vi "Tools Dialog.vi"(7 "Settings":T1, 8 "Error In":errorcluster, 10 "Context":refnum<k7>, 11 "Tools In":refnum<class "Tools.lvclass">[](array[class])) -> (0 "Error Out":errorcluster, 1 "Canceled?":bool, 2 "ID":string, 3 "Tools Out":refnum<class "Tools.lvclass">[](array[class]))   [LabVIEW 2021, in "Seq Edit Quick Drop.lvlib"]
uses:
  Seq Edit Quick Drop.lvlib
  Resources/Tool Menu Utility.lvlibp/Tools/Tools.lvclass
  Control Keys.ctl
  Get Modifier.vi
  <vilib>/addons/TestStand/_TSUtility.llb/TestStand - Start Modal Dialog (Sequence Context).vi
  <vilib>/Utility/error.llb/Trim Whitespace.vi
  <vilib>/addons/TestStand/_TSUtility.llb/TestStand - End Modal Dialog (Sequence Context).vi
panel:
  in  "Parameters":string
  in  "Tools":string(tree)
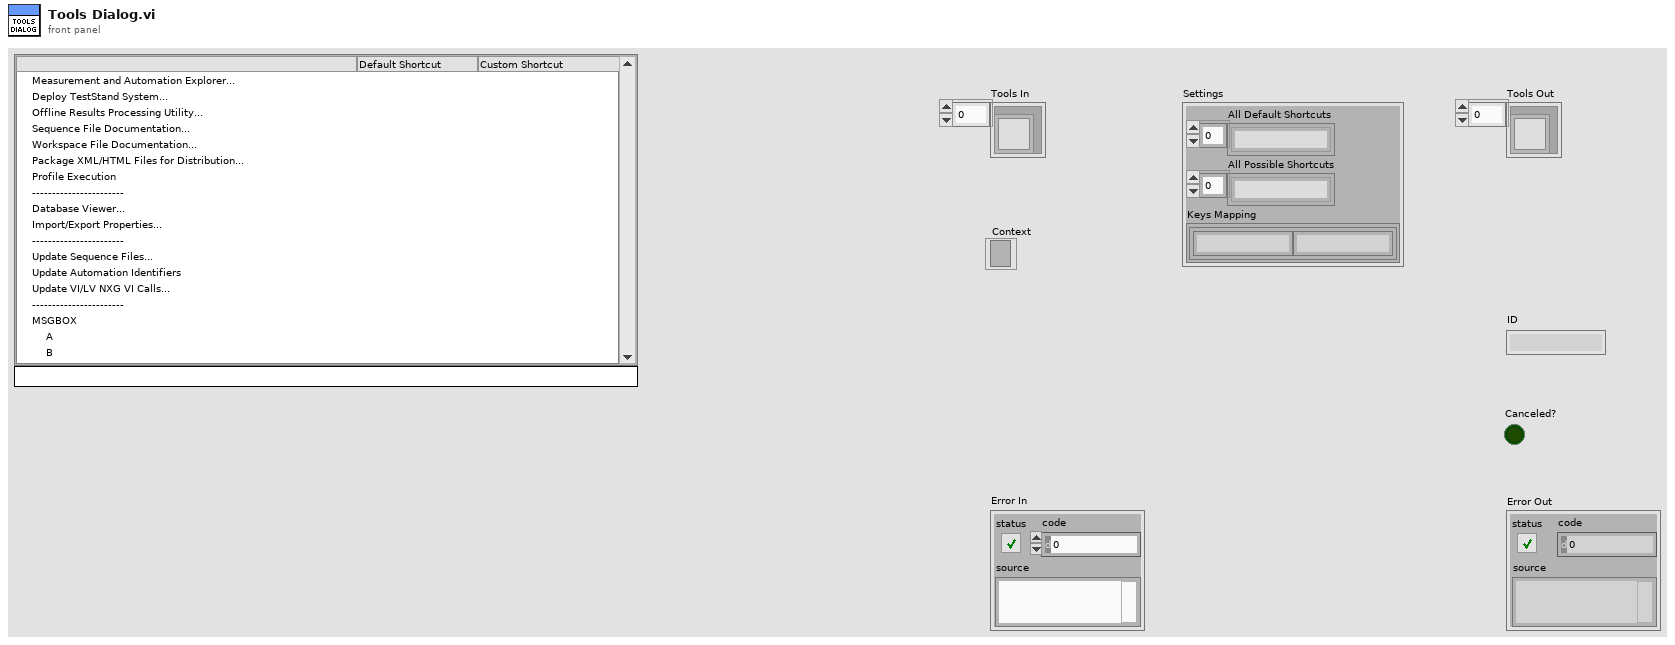
[diagram p1: front panel]
types:
  T1 = cluster{"All Default Shortcuts":string[], "All Possible Shortcuts":string[], "Keys Mapping":map{string, string}}
  T2 = typedef "Seq Edit Quick Drop.lvlib/Control Keys.ctl" = enum16{"Other", "Enter", "Escape", "Tab", "Up", "Down"}
  T3 = typedef "TestStand - Status Monitor.ctl" = cluster{"Sequence Context":refnum<k7>, "Execution":refnum<k7>, "Termination Monitor":refnum<k7>}
  T4 = cluster{"Shift":bool, "Ctrl":bool, "Alt":bool, "Cmd":bool, "Opt":bool}
  T5 = typedef "eventvkey.ctl" = enum16{"ASCII", "Enter", "Return", "Shift", "Ctrl", "Alt", "Cmd", "Opt", "Caps", "NumLock", "Clear", "Break", "Up", "Down", "Left", "Right", "Insert", "Delete", "Home", "End", "PageUp", "PageDown", "Escape", "Help", "Pause", "ScrollLock", "F1", "F2", "F3", "F4", "F5", "F6", "F7", "F8", "F9", "F10", "F11", "F12", "F13", "F14", "F15", "F16", "F17", "F18", "F19", "F20", "F21", "F22", "F23", "F24", "Play", "VolumeUp", "VolumeDown", "Mute", "Two Byte Char"}
  T6 = typedef "Seq Edit Quick Drop.lvlib/Modifiers.ctl" = enum16{"SHIFT", "CTRL", "ALT"}
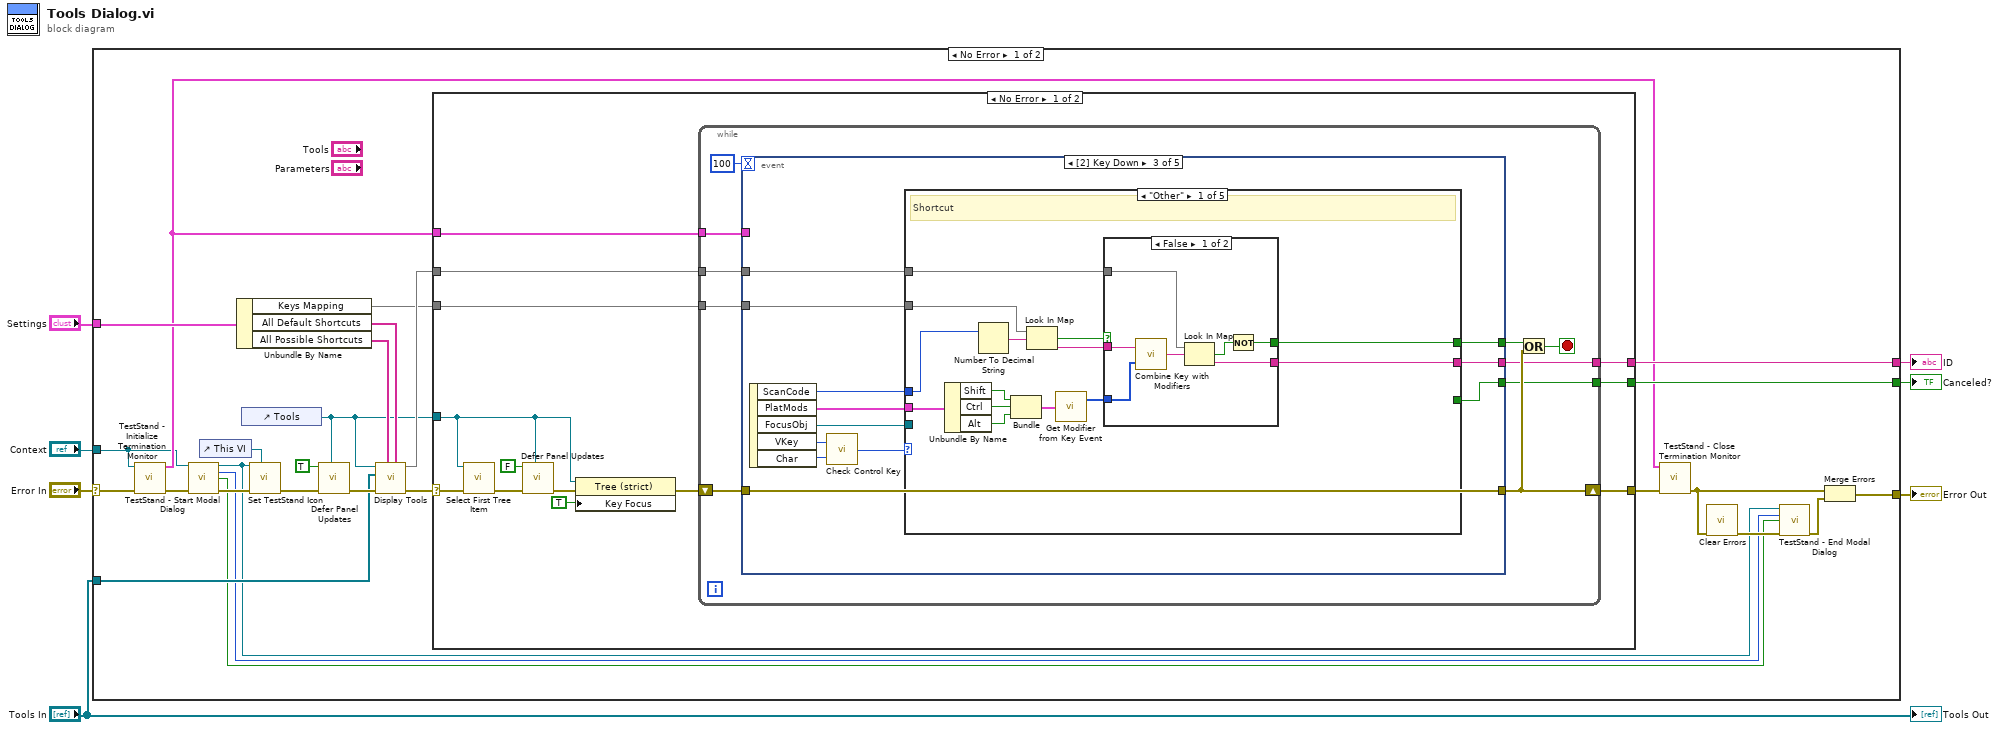
[diagram p0: block diagram]
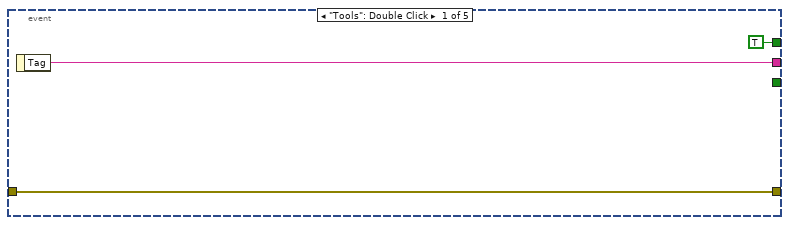
[diagram p2: hidden frame]
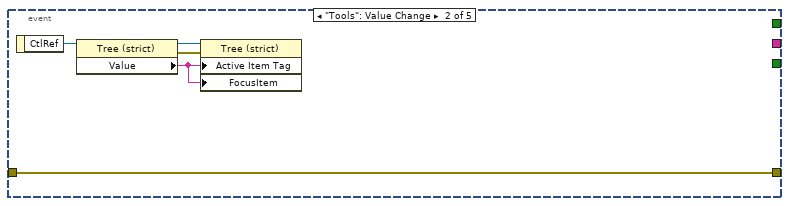
[diagram p3: hidden frame]
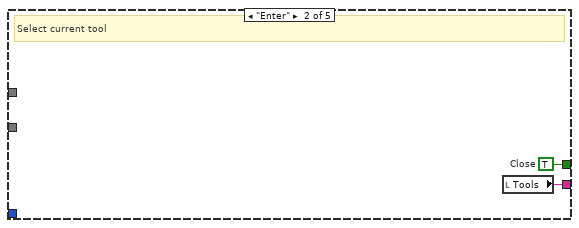
[diagram p5: hidden frame]
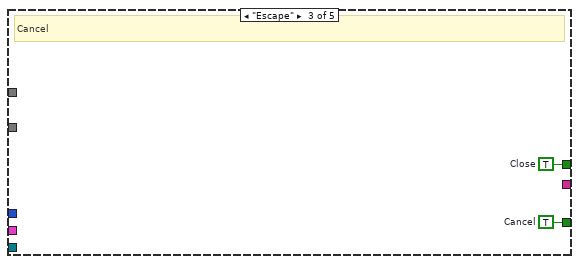
[diagram p6: hidden frame]
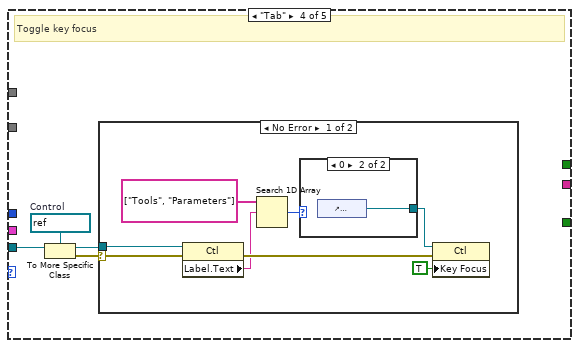
[diagram p7: hidden frame]
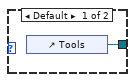
[diagram p8: hidden frame]
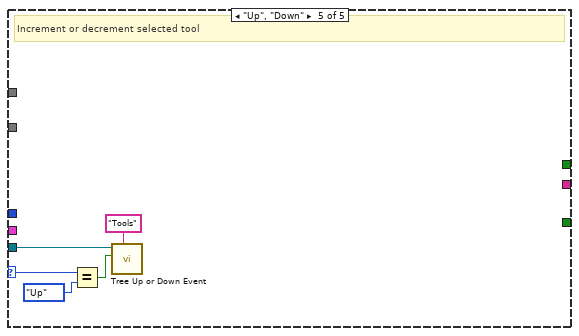
[diagram p10: hidden frame]
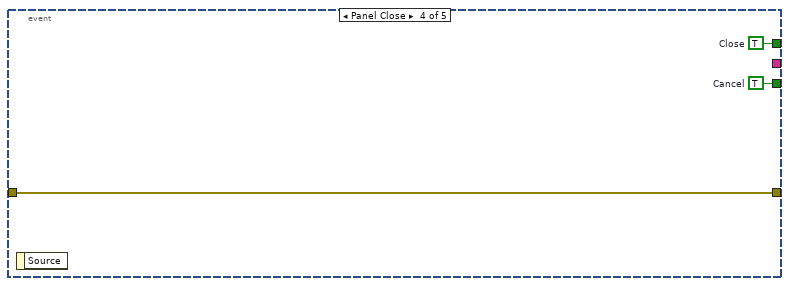
[diagram p11: hidden frame]
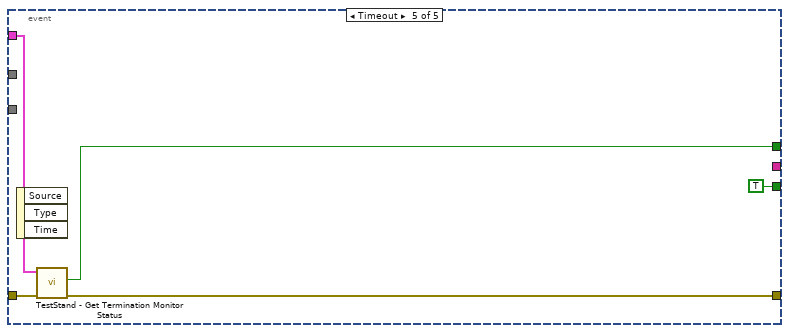
[diagram p12: hidden frame]
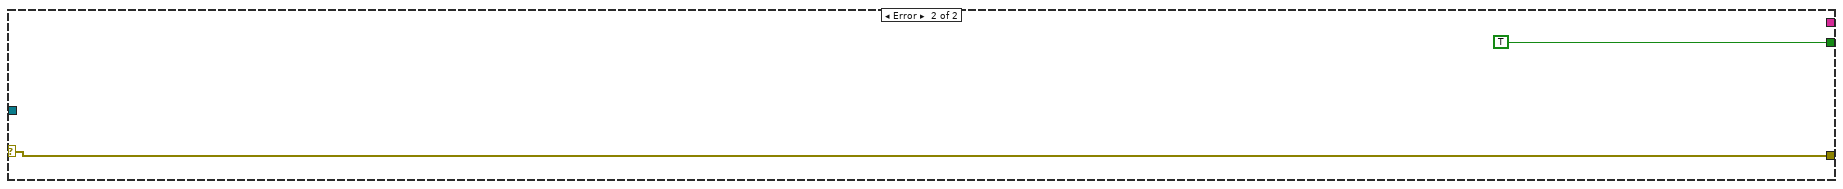
[diagram p14: hidden frame]
diagram:
  n1 = case shown="No Error" "Error In" {
    selector: "Error In" -> [w10 w132]
    tunnel: [w29 _] -> w7
    tunnel: "Tools In" -> [w28 _]
    tunnel: "Settings" -> [w27 _]
    tunnel: [w23 TRUE ("Cancel")] -> w4
    tunnel: [w21 w132] -> w3
    tunnel: "Context" -> [w12 _]
    frame No Error {
      n2 = call <vilib>:"TestStand - Initialize Termination Monitor.vi"("error in (no error)"=w10, "Sequence Context In"=w12) -> ("error out"=w18:errorcluster, "Status Monitor Out"=w16:T3)  [unwired: 8 in]
      n3 = call-poly <vilib>:"TestStand - Start Modal Dialog.vi"("Sequence Context In"=w12, "error in (no error)"=w18) -> ("Sequence Context Out"=w8:refnum<k7>, "Modal ID"=w20:i32, "VI Originally Open"=w19:bool, "error out"=w34:errorcluster)  [unwired: 9 in, 1 out]
      n4 = control-ref of="This VI"() -> (w9:refnum<vi>)
      n5 = Unbundle By Name(w27) -> ("Keys Mapping"=w24:map{string, string}, "All Default Shortcuts"=w25:string[], "All Possible Shortcuts"=w26:string[])
      n6 = control-ref of="Tools"() -> (w13:refnum<vi>)
      n7 = call "Set TestStand Icon.vi"("VI Reference"=w9, "Error In"=w34, "Context"=w8) -> ("Error Out"=w11:errorcluster)  [unwired: 8 in]
      n8 = call "Defer Panel Updates.vi"("Control"=w13, "Error In"=w11, "Defer Panel Updates"=TRUE) -> ("Error Out"=w31:errorcluster)  [unwired: 8 in]
      n9 = call "Display Tools.vi"("All Default Shortcuts"=w25, "All Possible Shortcuts"=w26, "Error In"=w31, "Tools"=w28, "Tools Tree Control"=w13) -> ("Error Out"=w32:errorcluster, "Shortcuts"=w30:map{string, string})  [unwired: 5 in]
      n10 = case shown="No Error" w32 {
        selector: w32 -> [w44 w130]
        tunnel: w30 -> [w46 _]
        tunnel: w13 -> [w38 _]
        tunnel: [w43 _] -> w29
        tunnel: w24 -> [w45 _]
        tunnel: [w42 _] -> w23
        tunnel: w16 -> [w36 _]
        tunnel: [w35 w130] -> w17
        frame No Error {
          n11 = call "Select First Tree Item.vi"("error in (no error)"=w44, "TreeControl in"=w38) -> ("error out"=w47:errorcluster)  [unwired: 8 in, 1 out]
          n12 = call "Defer Panel Updates.vi"("Control"=w38, "Error In"=w47, "Defer Panel Updates"=FALSE) -> ("Error Out"=w41:errorcluster)  [unwired: 8 in]
          n13 = property class="Tree (strict)"(reference=w38, error in=w41, "Key Focus"=TRUE) -> (error out=w39:errorcluster)  [unwired: 1 out]
          n14 = while {
            tunnel: [w56] -> w42
            tunnel: [w55] -> w43
            tunnel: w45 -> [w54]
            tunnel: w46 -> [w53]
            tunnel: w36 -> [w52]
            shift-right: [w57] -> w35
            shift-left: w39 -> [w50]
            stop <- w48 stop-if-true
            n15 = event shown="[2] Key Down" {
              selector: _ -> [_ _ _ _ _]
              dyn-events: _ -> [_ _ _ _ _]
              timeout: 100 -> [_ _ _ _ _]
              tunnel: [_ _ w72 w124 TRUE ("Cancel")] -> w56
              tunnel: [w60 _ w73 _ _] -> w55
              tunnel: w54 -> [_ _ w76 _ _]
              tunnel: [TRUE ("Close") _ w71 w123 w129] -> w49
              tunnel: w53 -> [_ _ w70 _ _]
              tunnel: w52 -> [_ _ _ _ w127]
              tunnel: w50 -> [w58 w61 w66 w122 w126]
              tunnel: [w58 w61 w66 w122 w125] -> w57
              event "Tools": Double Click {
                n16 = event-data() -> ("Tag"=w60:string)  [unwired: 1 in]
              }
              event "Tools": Value Change {
                n17 = event-data() -> ("CtlRef"=w65:refnum<vi>)  [unwired: 1 in]
                n18 = property class="Tree (strict)"(reference=w65) -> (reference out=w64:refnum<vi>, error out=w63:errorcluster, "Value"=w62:string)  [unwired: 1 in]
                n19 = property class="Tree (strict)"(reference=w64, error in=w63, "Active Item Tag"=w62, "FocusItem"=w62) -> ()  [unwired: 2 out]
              }
              event Key Down {
                n20 = event-data() -> ("ScanCode"=w77:i16, "PlatMods"=w75:T4, "FocusObj"=w67:refnum<vi>, "VKey"=w68:T5, "Char"=w69:i16)  [unwired: 1 in]
                n21 = call "Check Control Key.vi"("Char"=w69, "VKey"=w68) -> ("Control Key"=w74:T2)
                n22 = case shown="\"Other\"" w74 {
                  selector: w74 -> [_ _ _ _ w119]
                  tunnel: w77 -> [w91 _ _ _ _]
                  tunnel: w76 -> [w89 _ _ _ _]
                  tunnel: w75 -> [w85 _ _ _ _]
                  tunnel: [w79 w100 _ _ _] -> w73
                  tunnel: [_ _ w102 _ _] -> w72
                  tunnel: [w78 w99 w101 _ _] -> w71
                  tunnel: w67 -> [_ _ _ w106 w121]
                  tunnel: w70 -> [w80 _ _ _ _]
                  frame "Other" {
                    # "Shortcut"
                    n23 = Unbundle By Name(w85) -> ("Shift"=w84:bool, "Ctrl"=w83:bool, "Alt"=w82:bool)
                    n24 = Number To Decimal String(number=w91) -> (decimal integer string=w90:string)  [unwired: 1 in]
                    n25 = Bundle("Shift"=w84, "Ctrl"=w83, "Alt"=w82) -> (w81:cluster{"Shift":bool, "Ctrl":bool, "Alt":bool})  [unwired: 1 in]
                    n26 = Look In Map(map=w89, key=w90) -> (key not found?=w88:bool, value=w86:string)  [unwired: 1 in]
                    n27 = call "Get Modifier from Key Event.vi"("Modifiers"=w81) -> ("Modifiers"=w87:T6[])  [unwired: 1 out]
                    n28 = case shown="False" w88 {
                      tunnel: w87 -> [w98 _]
                      tunnel: w86 -> [w97 _]
                      tunnel: w80 -> [w95 _]
                      tunnel: [w94 _] -> w79
                      tunnel: [w92 _] -> w78
                      frame False {
                        n29 = call "Combine Key with Modifiers.vi"("Modifiers"=w98, "Key"=w97) -> ("Combined"=w96:string)
                        n30 = Look In Map(map=w95, key=w96) -> (key not found?=w93:bool, value=w94:string)  [unwired: 1 in]
                        n31 = Not(x=w93) -> (.not. x?=w92:bool)
                      }
                      frame True {
                      }
                    }
                  }
                  frame "Enter" {
                    w99 = TRUE  # Close
                    # "Select current tool"
                    n32 = local read "Tools"() -> (w100:string)
                  }
                  frame "Escape" {
                    w101 = TRUE  # Close
                    w102 = TRUE  # Cancel
                    # "Cancel"
                  }
                  frame "Tab" {
                    w105 = refnum<vi> refnum  # Control
                    # "Toggle key focus"
                    n33 = To More Specific Class(target class=w105, reference=w106) -> (specific class reference=w103:refnum<vi>, error out=w104:errorcluster)  [unwired: 1 in]
                    n34 = case shown="No Error" w104 {
                      selector: w104 -> [w112 _]
                      tunnel: w103 -> [w113 _]
                      frame No Error {
                        n35 = property class="Ctl"(reference=w113, error in=w112) -> (error out=w114:errorcluster, "Label.Text"=w111:string)  [unwired: 1 out]
                        n36 = Search 1D Array(1D array=string[] ["Tools", "Parameters"], element=w111) -> (index of element=w109:i32)  [unwired: 1 in]
                        n37 = case shown="0" w109 {
                          tunnel: [w115 w116] -> w108
                          frame Default {
                            n38 = control-ref of="Tools"() -> (w115:refnum<vi>)
                          }
                          frame 0 {
                            n39 = control-ref of="Parameters"() -> (w116:refnum<vi>)
                          }
                        }
                        n40 = property class="Ctl"(reference=w108, error in=w114, "Key Focus"=TRUE) -> ()  [unwired: 2 out]
                      }
                      frame Error {
                      }
                    }
                  }
                  frame "Up", "Down" {
                    # "Increment or decrement selected tool"
                    n41 = Equal?(x=w119, y=Control_Keys."Up") -> (x = y?=w117:bool)
                    n42 = call "Tree Up or Down Event.vi"("Label"="Tools", "Up?"=w117, "GObject"=w121) -> ()  [unwired: 9 in]
                  }
                }
              }
              event Panel Close {
                w123 = TRUE  # Close
                w124 = TRUE  # Cancel
                n43 = event-data() -> ()  [unwired: 1 in, 1 out]
              }
              event Timeout {
                n44 = event-data() -> ()  [unwired: 1 in, 3 out]
                n45 = call <vilib>:"TestStand - Get Termination Monitor Status.vi"("error in (no error)"=w126, "Status Monitor In"=w127) -> ("error out"=w125:errorcluster, "Terminating or Aborting"=w129:bool)  [unwired: 7 in, 1 out]
              }
            }
            n46 = Or(x=w49, y=w57) -> (x .or. y?=w48:bool)
          }
        }
        frame Error {
        }
      }
      n47 = call <vilib>:"TestStand - Close Termination Monitor.vi"("error in (no error)"=w17, "Status Monitor In"=w16) -> ("error out"=w15:errorcluster)  [unwired: 9 in]
      n48 = call <vilib>:"Clear Errors.vi"("error in (no error)"=w15) -> ("error out"=w33:errorcluster)  [unwired: 5 in, 1 out]
      n49 = call-poly <vilib>:"TestStand - End Modal Dialog.vi"("Sequence Context In"=w8, "Modal ID"=w20, "VI Originally Open"=w19, "error in (no error)"=w33) -> ("error out"=w14:errorcluster)  [unwired: 11 in]
      n50 = Merge Errors(w15, w14) -> (w21:errorcluster)
    }
    frame Error {
    }
  }
  "Error Out" <- w3
  "Canceled?" <- w4
  "ID" <- w7
  "Tools Out" <- "Tools In"
